vi "Test Threaded Parallel.vi"() -> ()   [LabVIEW 2021]
uses:
  Source/Blackboard/Blackboard.lvclass
  Source/Support/Nodes/Decorators/Repeater/Support/Finish On - Type.ctl
  Source/Blackboard/Blackboard.lvclass/Blackboard.ctl
  Source/Support/Nodes/Leaves/abs_Type Leaf/abs_Type Leaf.lvclass/abs_Type Leaf.ctl
  Source/Support/Nodes/Composites/abs_Parallel/Support/Status Calculation.ctl
  Source/System/bt_System.lvclass/bt_System.ctl
  Source/Blackboard/Get Value Type/Get I32.vi
  <vilib>/TSA/Abstract Data Classes/Abs_Types/I32 Integer/Static Read.vi
  Source/System/Properties/Write Behaviour Tree.vi
  Source/Blackboard/Support/Index Group.vi
  Source/Blackboard/Support/Index Tags.vi
  Source/Support/Nodes/Leaves/abs_Type Leaf/Properties/Write Value Class.vi
  <vilib>/TSA/Abstract Data Classes/Abs_Types/I32 Integer/Abs_I32 Integer.lvclass
  C:/Program Files (x86)/National Instruments/LabVIEW 2021/vi.lib/TSA/Abstract Data Classes/Abs_Types/Numeric/Abs_Numeric.lvclass
  C:/Program Files (x86)/National Instruments/LabVIEW 2021/vi.lib/TSA/Abstract Data Classes/Abs_Types/Value/Abs_Value.lvclass
  <vilib>/TSA/Omni-Bus/Local Bus/Support/I32/Local Bus_I32.lvclass
  Source/Support/Nodes/Leaves/Test Boolean/Test Abs_Boolean.lvclass
  C:/Users/Tim/Documents/GitHub/LV_Behaviour_Tree/Source/Support/Nodes/abs_Node/bt_Node.lvclass
  C:/Users/Tim/Documents/GitHub/LV_Behaviour_Tree/Source/Support/Nodes/Leaves/abs_Type Leaf/abs_Type Leaf.lvclass
  <vilib>/TSA/Abstract Data Classes/Abs_Types/Boolean/Abs_Boolean.lvclass
  C:/Program Files (x86)/National Instruments/LabVIEW 2021/vi.lib/TSA/Abstract Data Classes/Abs_Types/Type/Abs_Type.lvclass
  <vilib>/TSA/Omni-Bus/Local Bus/Support/Initialise DVR's.vi
  <vilib>/TSA/Abstract Data Classes/Functions/Math/Support/Increment/I32/Method.vi
  <vilib>/TSA/Abstract Data Classes/Constants/Support/I32/I32.vi
  <vilib>/TSA/Abstract Data Classes/Functions/Math/Support/Add/I32/Method.vi
  <vilib>/TSA/Abstract Data Classes/Functions/Compare/Support/Less/I32/Method.vi
  <vilib>/TSA/Abstract Data Classes/Abs_Types/Value/Abs_Value.lvclass
  <vilib>/TSA/Abstract Data Classes/Abs_Types/Type/Abs_Type.lvclass
  <vilib>/TSA/Omni-Bus/Local Bus/Support/DBL/Local Bus_DBL.lvclass
  <vilib>/TSA/Omni-Bus/Local Bus/Support/SGL/Local Bus_SGL.lvclass
  <vilib>/TSA/Omni-Bus/Local Bus/Support/EXT/Local Bus_EXT.lvclass
  <vilib>/TSA/Omni-Bus/Local Bus/Support/Bool/Local Bus_Boolean.lvclass
  <vilib>/TSA/Omni-Bus/Local Bus/Support/STR/Local Bus_String.lvclass
  <vilib>/TSA/Omni-Bus/Local Bus/Support/Variant/Local Bus_Variant.lvclass
  <vilib>/TSA/Omni-Bus/Local Bus/Support/WFM/Local Bus_Waveform.lvclass
  <vilib>/TSA/Omni-Bus/Local Bus/Support/Time/Local Bus_Time.lvclass
  <vilib>/TSA/Omni-Bus/Local Bus/Support/U8/Local Bus_U8.lvclass
  <vilib>/TSA/Omni-Bus/Local Bus/Support/U16/Local Bus_U16.lvclass
  <vilib>/TSA/Omni-Bus/Local Bus/Support/U32/Local Bus_U32.lvclass
  <vilib>/TSA/Omni-Bus/Local Bus/Support/U64/Local Bus_U64.lvclass
  <vilib>/TSA/Omni-Bus/Local Bus/Support/I8/Local Bus_I8.lvclass
  <vilib>/TSA/Omni-Bus/Local Bus/Support/I16/Local Bus_I16.lvclass
  <vilib>/TSA/Omni-Bus/Local Bus/Support/I64/Local Bus_I64.lvclass
  <vilib>/TSA/Omni-Bus/Local Bus/Support/CSGL/Local Bus_CSGL.lvclass
  <vilib>/TSA/Omni-Bus/Local Bus/Support/CDBL/Local Bus_CDBL.lvclass
  <vilib>/TSA/Omni-Bus/Local Bus/Support/CEXT/Local Bus_CEXT.lvclass
  Source/BT.lvlib
  Source/Support/Nodes/Decorators/Repeater/bt_Repeater.lvclass
  Source/Support/Nodes/Composites/abs_Parallel/bt_Parallel.lvclass
  C:/Program Files (x86)/National Instruments/LabVIEW 2021/vi.lib/TSA/Abstract Data Classes/Abs_Types/Integer/Abs_Integer.lvclass
  C:/Program Files (x86)/National Instruments/LabVIEW 2021/vi.lib/TSA/Abstract Data Classes/Abs_Types/I32 Integer/Abs_I32 Integer.lvclass
  <vilib>/TSA/Abstract Data Classes/Constants/Support/I32/Const_I32.lvclass
  <vilib>/TSA/Abstract Data Classes/Functions/Compare/Support/Less/I32/Less_I32.lvclass
  <vilib>/TSA/Abstract Data Classes/Functions/Math/Support/Increment/I32/Increment_I32.lvclass
  Source/System/bt_System.lvclass
  <vilib>/TSA/Abstract Data Classes/Functions/Math/Support/Add/I32/Add_I32.lvclass
panel:
  out "Counts":i32[](array[numeric])
  in  "stop":bool
  # "Count 1"
  # "Count 2"
  # "Finish Count"
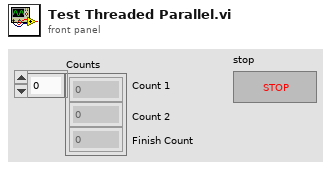
[diagram p1: front panel]
types:
  T1 = typedef "BT.lvlib/bt_Repeater.lvclass/Finish On - Type.ctl" = enum16{"Success", "Failure", "Never"}
  T2 = typedef "Add_I32.lvclass/Abs_Type.ctl" = refnum<class "Abs_I32 Integer.lvclass">
  T3 = typedef "BT.lvlib/bt_Parallel.lvclass/Status Calculation.ctl" = enum16{"Succeed on All Succeed", "Failure on All Failure", "Succeed on Any Succeed", "Failure on Any Failure"}
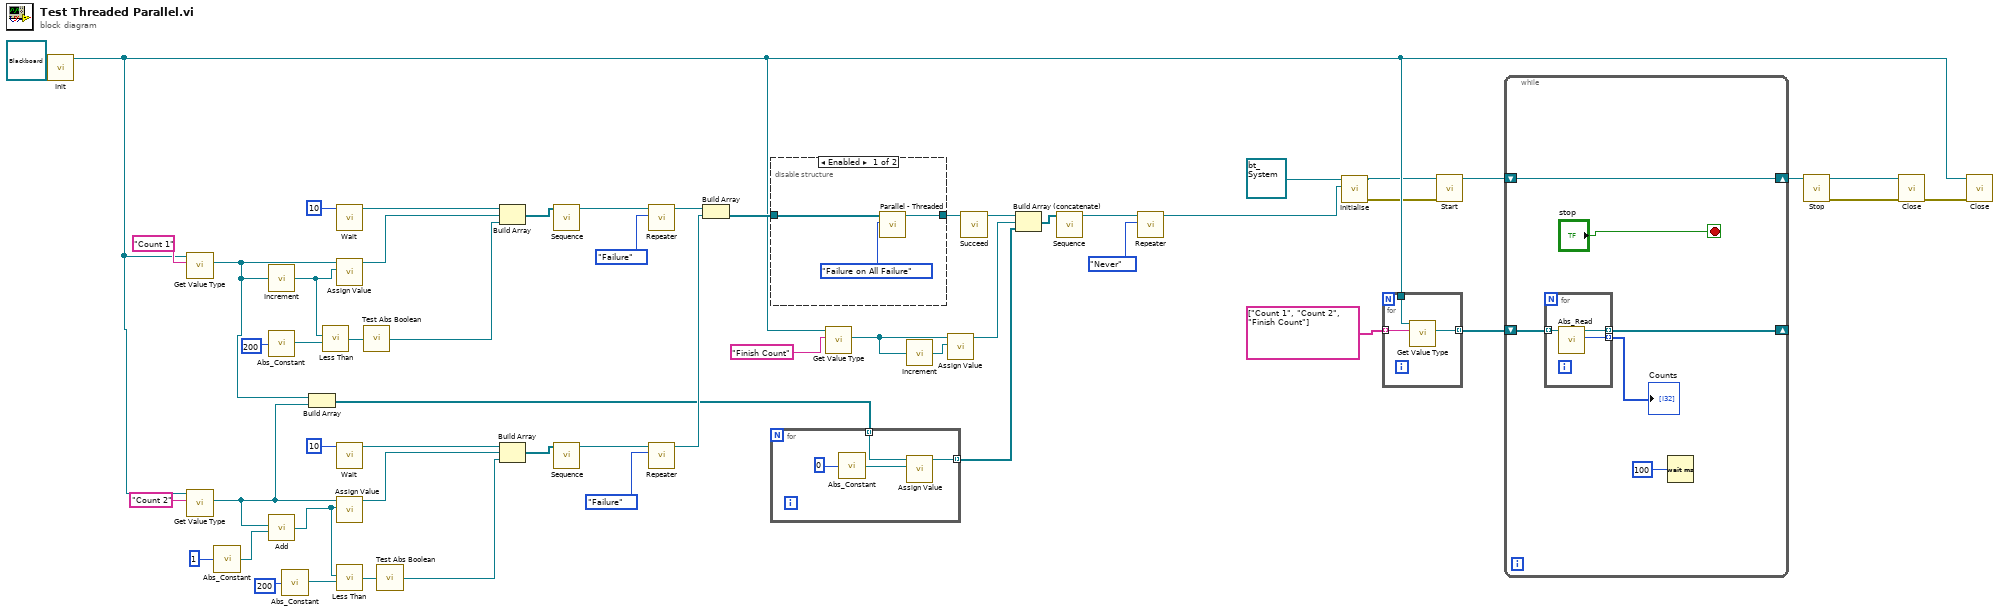
[diagram p0: block diagram]
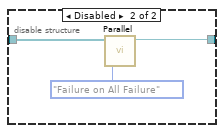
[diagram p2: hidden frame]
diagram:
  n1 = call-dynamic "Init.vi"("bt_Blackboard in"=refnum<class "Blackboard.lvclass"> refnum) -> ("bt_Blackboard out"=w16:refnum<class "Blackboard.lvclass">)  [unwired: 9 in, 1 out]
  n2 = call-poly "Get Value Type.vi"("Tag"="Count 1", "Blackboard in"=w16) -> ("Value"=w9:refnum<class "Abs_I32 Integer.lvclass">)  [unwired: 6 in, 3 out]
  n3 = call-poly "Get Value Type.vi"("Tag"="Count 2", "Blackboard in"=w16) -> ("Value"=w8:refnum<class "Abs_I32 Integer.lvclass">)  [unwired: 6 in, 3 out]
  n4 = call-poly <vilib>:"Abs_Constant.vi"("Value"=1) -> ("Constant"=w39:refnum<class "Abs_I32 Integer.lvclass">)  [unwired: 4 in]
  n5 = call-poly <vilib>:"Increment.vi"("Value"=w9) -> ("Result"=w24:refnum<class "Abs_I32 Integer.lvclass">)  [unwired: 4 in]
  n6 = call-poly <vilib>:"Abs_Constant.vi"("Value"=200) -> ("Constant"=w25:refnum<class "Abs_I32 Integer.lvclass">)  [unwired: 4 in]
  n7 = call-poly <vilib>:"Add.vi"("Input B"=w39, "Input A"=w8) -> ("Result"=w31:T2)  [unwired: 4 in]
  n8 = call-poly <vilib>:"Abs_Constant.vi"("Value"=200) -> ("Constant"=w30:refnum<class "Abs_I32 Integer.lvclass">)  [unwired: 4 in]
  n9 = Build Array(w9, w8) -> (w7:refnum<class "Abs_I32 Integer.lvclass">[])
  n10 = call-poly <vilib>:"Less Than.vi"("Value B"=w25, "Value A"=w24) -> ("Result"=w27:refnum<class "Abs_Boolean.lvclass">)  [unwired: 4 in]
  n11 = call "Wait.vi"("Time (ms)"=u32 10) -> ("Node Out"=w53:refnum<class "bt_Node.lvclass">)  [unwired: 10 in]
  n12 = call "Assign Value.vi"("Assigned Value"=w24, "Value"=w9) -> ("Node Out"=w47:refnum<class "bt_Node.lvclass">)  [unwired: 9 in]
  n13 = call "Wait.vi"("Time (ms)"=u32 10) -> ("Node Out"=w40:refnum<class "bt_Node.lvclass">)  [unwired: 10 in]
  n14 = call "Assign Value.vi"("Assigned Value"=w31, "Value"=w8) -> ("Node Out"=w43:refnum<class "bt_Node.lvclass">)  [unwired: 9 in]
  n15 = call-poly <vilib>:"Less Than.vi"("Value B"=w30, "Value A"=w31) -> ("Result"=w28:refnum<class "Abs_Boolean.lvclass">)  [unwired: 4 in]
  n16 = call "Test Abs Boolean.vi"("Abs_Boolean.lvclass"=w27) -> ("abs_Node"=w10:refnum<class "bt_Node.lvclass">)  [unwired: 4 in]
  n17 = call "Test Abs Boolean.vi"("Abs_Boolean.lvclass"=w28) -> ("abs_Node"=w12:refnum<class "bt_Node.lvclass">)  [unwired: 4 in]
  n18 = Build Array(w53, w47, w10) -> (w52:refnum<class "bt_Node.lvclass">[])
  n19 = Build Array(w40, w43, w12) -> (w41:refnum<class "bt_Node.lvclass">[])
  n20 = call "Sequence.vi"("Nodes"=w52) -> ("Node"=w37:refnum<class "bt_Node.lvclass">)  [unwired: 10 in]
  n21 = call "Sequence.vi"("Nodes"=w41) -> ("Node"=w33:refnum<class "bt_Node.lvclass">)  [unwired: 10 in]
  n22 = call "Repeater.vi"("Finish On"=Finish_On_-_Type."Failure", "Node In"=w37) -> ("Node Out"=w36:refnum<class "bt_Node.lvclass">)  [unwired: 9 in]
  n23 = call "Repeater.vi"("Finish On"=Finish_On_-_Type."Failure", "Node In"=w33) -> ("Node Out"=w32:refnum<class "bt_Node.lvclass">)  [unwired: 9 in]
  n24 = Build Array(w36, w32) -> (w23:refnum<class "bt_Node.lvclass">[])
  n25 = disable-structure shown="Enabled" {
    disable-tunnel: w23 -> [w57 w61]
    disable-tunnel: [w56 w60] -> w15
    frame Enabled {
      n26 = call "Parallel - Threaded.vi"("Status Calculation"=Status_Calculation."Failure on All Failure", "Nodes"=w57) -> ("Node"=w56:refnum<class "bt_Node.lvclass">)  [unwired: 9 in]
    }
    frame Disabled {
      n27 = call "Parallel.vi"("Status Calculation"=Status_Calculation."Failure on All Failure", "Nodes"=w61) -> ("Node"=w60:refnum<class "bt_Node.lvclass">)  [unwired: 9 in]
    }
  }
  n28 = for {
    tunnel: [w63] -> w11 mode=indexing
    tunnel: w7 -> [w62] mode=indexing
    n29 = call-poly <vilib>:"Abs_Constant.vi"("Value"=0) -> ("Constant"=w64:refnum<class "Abs_I32 Integer.lvclass">)  [unwired: 4 in]
    n30 = call "Assign Value.vi"("Assigned Value"=w64, "Value"=w62) -> ("Node Out"=w63:refnum<class "bt_Node.lvclass">)  [unwired: 9 in]
  }
  n31 = call-poly "Get Value Type.vi"("Tag"="Finish Count", "Blackboard in"=w16) -> ("Value"=w21:refnum<class "Abs_I32 Integer.lvclass">)  [unwired: 6 in, 3 out]
  n32 = call-poly <vilib>:"Increment.vi"("Value"=w21) -> ("Result"=w20:refnum<class "Abs_I32 Integer.lvclass">)  [unwired: 4 in]
  n33 = call "Assign Value.vi"("Assigned Value"=w20, "Value"=w21) -> ("Node Out"=w13:refnum<class "bt_Node.lvclass">)  [unwired: 9 in]
  n34 = call "Succeed.vi"("Node In"=w15) -> ("Node"=w14:refnum<class "bt_Node.lvclass">)  [unwired: 10 in]
  n35 = Build Array (concatenate)(w14, w13, w11) -> (w18:refnum<class "bt_Node.lvclass">[])
  n36 = call "Sequence.vi"("Nodes"=w18) -> ("Node"=w17:refnum<class "bt_Node.lvclass">)  [unwired: 10 in]
  n37 = call "Repeater.vi"("Finish On"=Finish_On_-_Type."Never", "Node In"=w17) -> ("Node Out"=w1:refnum<class "bt_Node.lvclass">)  [unwired: 9 in]
  n38 = call "Initialise.vi"("Behaviour Tree"=w1, "bt_System in"=refnum<class "bt_System.lvclass"> refnum ("BT.lvlib:bt_System.lvclass")) -> ("error out"=w3:errorcluster, "bt_System out"=w4:refnum<class "bt_System.lvclass">)  [unwired: 8 in]
  n39 = for {
    tunnel: string[] ["Count 1", "Count 2", "Finish Count"] ("Tag") -> [w68] mode=indexing
    tunnel: [w67] -> w45 mode=indexing
    tunnel: w16 -> [w66]
    n40 = call-poly "Get Value Type.vi"("Tag"=w68, "Blackboard in"=w66) -> ("Value"=w67:refnum<class "Abs_I32 Integer.lvclass">)  [unwired: 6 in, 3 out]
  }
  n41 = call "Start.vi"("error in (no error)"=w3, "bt_System in"=w4) -> ("bt_System out"=w55:refnum<class "bt_System.lvclass">)  [unwired: 8 in, 1 out]
  n42 = while {
    shift-right: [w71] -> w54
    shift-left: w55 -> [w71]
    shift-right: [w73] -> _
    shift-left: w45 -> [w74]
    stop <- "stop" stop-if-true
    n43 = for {
      tunnel: w74 -> [w77] mode=indexing
      tunnel: [w76] -> w73 mode=indexing
      tunnel: [w75] -> w72 mode=indexing
      n44 = call-poly <vilib>:"Abs_Read.vi"("Abs_I32 Integer in"=w77) -> ("Value"=w75:i32, "Abs_I32 Integer out"=w76:refnum<class "Abs_I32 Integer.lvclass">)  [unwired: 8 in, 1 out]
    }
    "Counts" <- w72
    n45 = Wait (ms)(milliseconds to wait=u32 100) -> ()  [unwired: 1 out]
  }
  n46 = call "Stop.vi"("bt_System in"=w54) -> ("error out"=w5:errorcluster, "bt_System out"=w6:refnum<class "bt_System.lvclass">)  [unwired: 9 in]
  n47 = call-dynamic "Close.vi"("error in (no error)"=w5, "bt_System in"=w6) -> ("error out"=w50:errorcluster)  [unwired: 8 in, 1 out]
  n48 = call-dynamic "Close.vi"("error in (no error)"=w50, "bt_Blackboard in"=w16) -> ()  [unwired: 8 in, 2 out]
